vi "Command.vi"(8 "error in (no error)":errorcluster, 11 "Node Ptr":T1 format="%.0x") -> (0 "error out":errorcluster)   [LabVIEW 2020, in "Instrument Addon System Explorer.lvlib"]
uses:
  Instrument Addon System Explorer.lvlib
  <vilib>/NI VeriStand/Custom Device API/Custom Device API.lvlib
  Addon Shared/Instrument Addon Shared.lvlib
  Addon Shared/Types/FG Control.ctl
  <vilib>/NI VeriStand/Custom Device API/Custom Device Item Ref.ctl
panel:
  in  "Pad Value":u8=32 format="%.0x"
  in  "Length":u32=25 caption="Length (Bytes)"
  in  "Pad":bool caption="Pad?"
  in  "Linkages":i32(listbox)
  in  "MetaData":string(combo) caption="Available MetaData Channels"
  in  "Command":string caption="Command ( Use [] to define a variable )"
  in  "Header 2":cluster{"Section Name":string}={"Section Name"="Command Message Settings"}
  in  "SHDocVw.IWebBrowser":refnum<k7>(container)
  in  "Header":cluster{"Section Name":string}={"Section Name"="Command Settings"}
  in  "Description":string
  out "Name":string
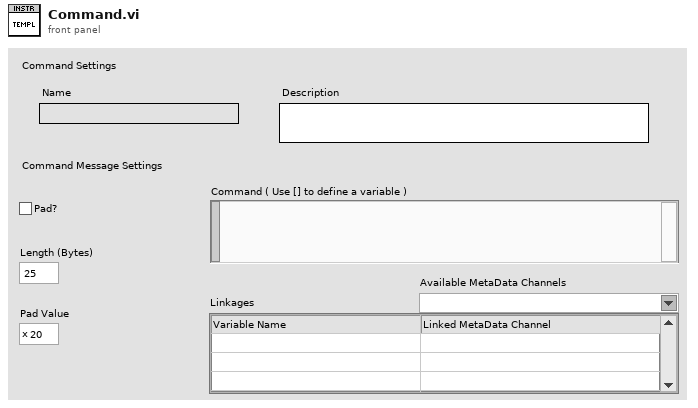
[diagram p1: front panel]
types:
  T1 = typedef "Custom Device API.lvlib/Custom Device Item Ref.ctl" = u64
  T2 = typedef "Instrument Addon Shared.lvlib/FG Control.ctl" = enum16{"Get", "Set"}
  T3 = typedef "Instrument Addon Shared.lvlib/Command Parameters.ctl" = cluster{"Command":string, "Linked Channels":T4[], "Pad":bool, "Length":u32, "Pad Value":u8}
  T4 = typedef "Instrument Addon Shared.lvlib/Linked Channel Cluster.ctl" = cluster{"Variable Name":string, "GUID":string}
  T5 = typedef "Custom Device API.lvlib/Custom Device Item Info.ctl" = cluster{"Name":string, "Is Channel":bool, "GUID":string, "Is Waveform":bool}
  T6 = typedef "Custom Device API.lvlib/Custom Device Commands.ctl" = enum16{"Default", "Item renamed", "Shutdown", "Dynamic button pressed"}
  T7 = typedef "LVComboBoxStrsAndValuesArrayTypeDef.ctl" = cluster{"String":string, "Value":string}[]
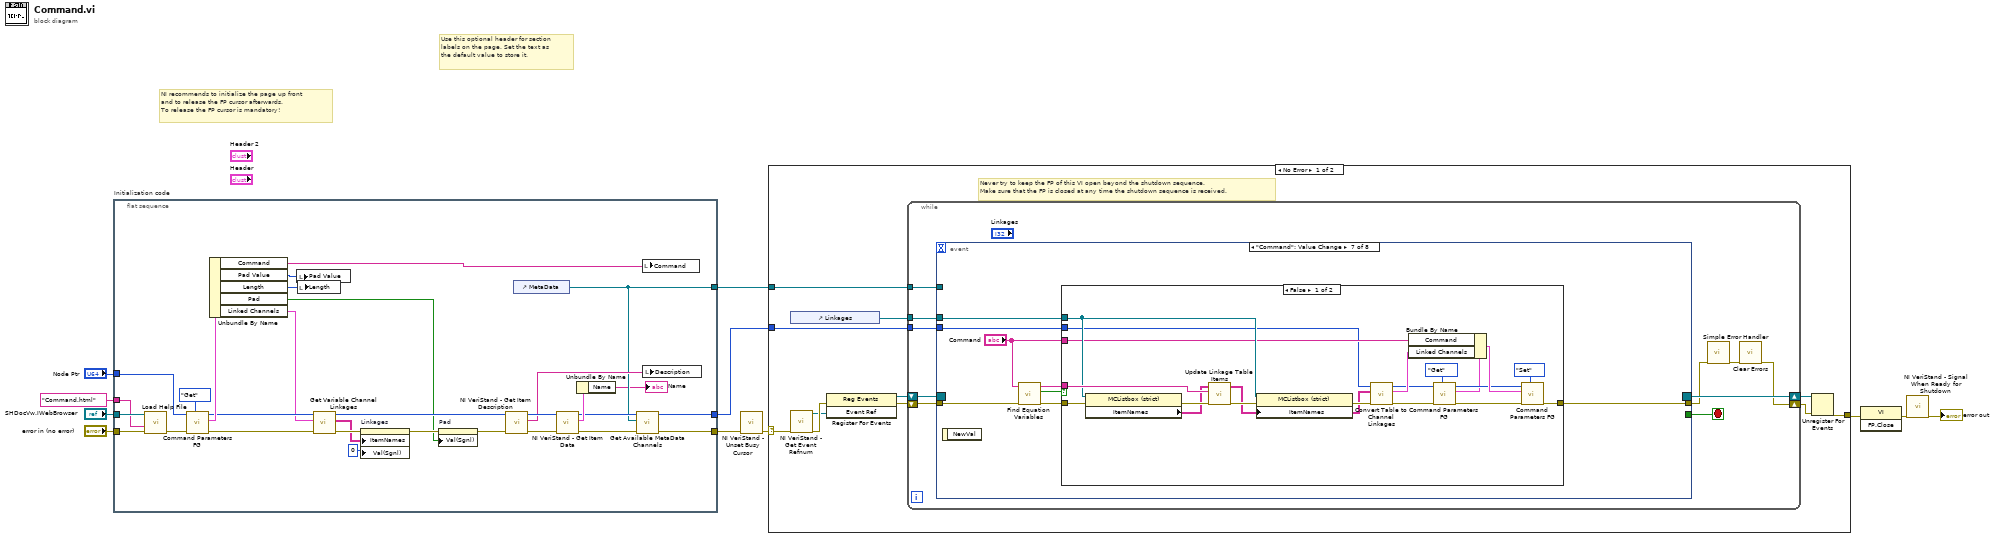
[diagram p0: block diagram]
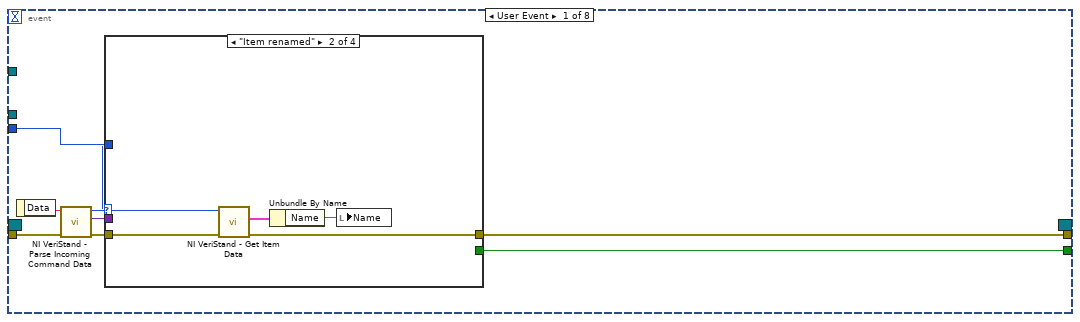
[diagram p2: hidden frame]
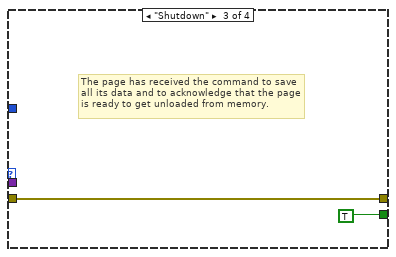
[diagram p4: hidden frame]
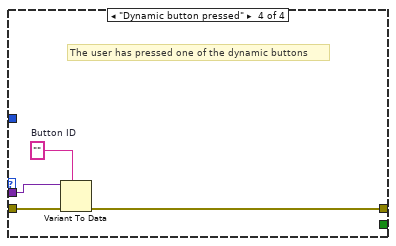
[diagram p5: hidden frame]
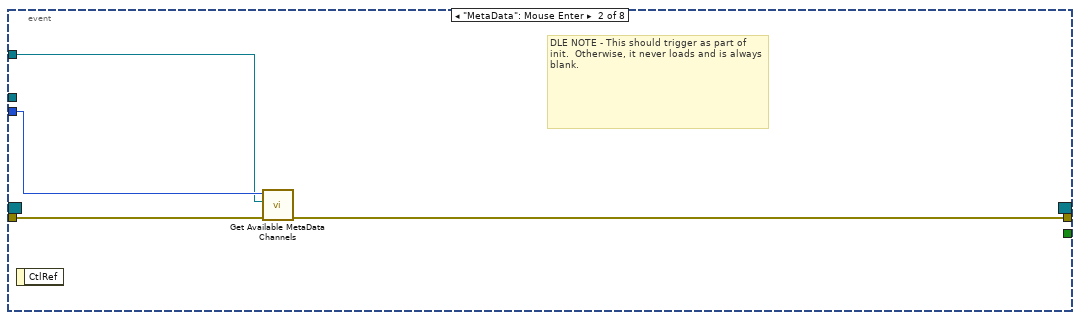
[diagram p6: hidden frame]
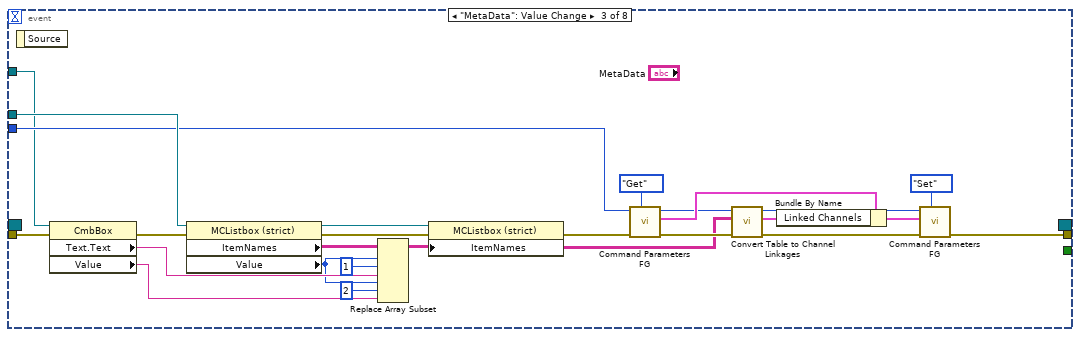
[diagram p7: hidden frame]
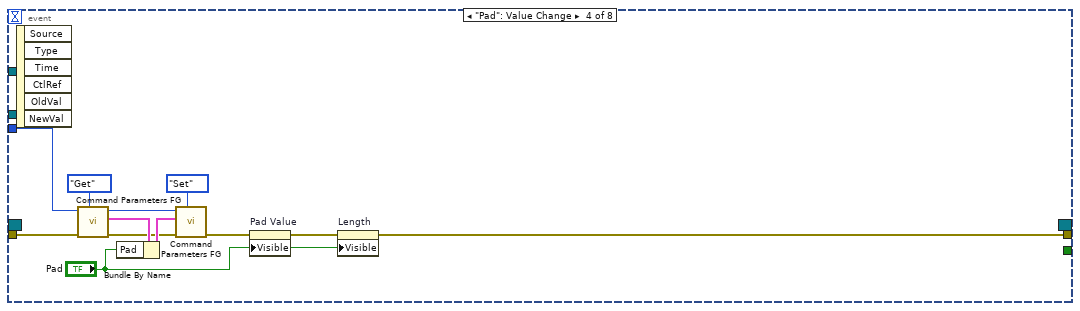
[diagram p8: hidden frame]
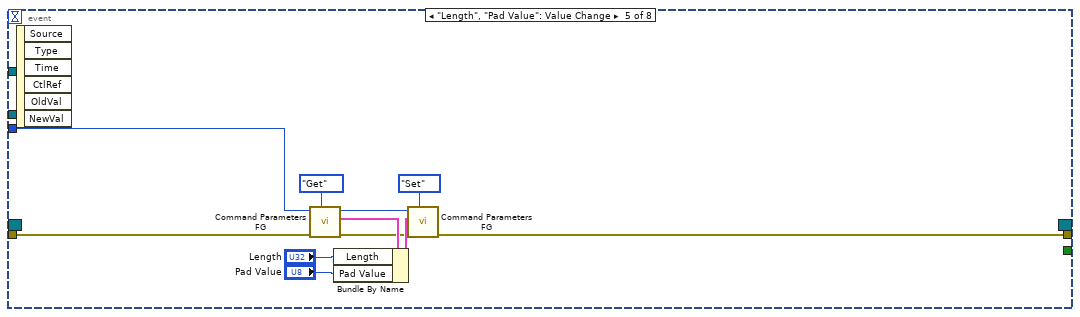
[diagram p9: hidden frame]
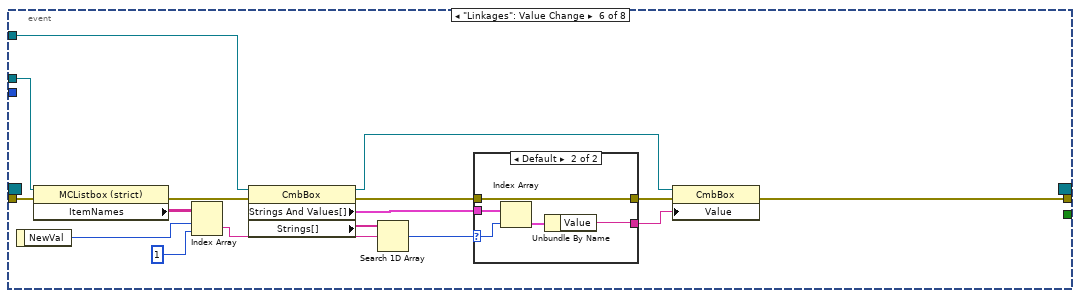
[diagram p10: hidden frame]
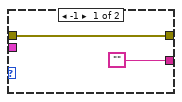
[diagram p11: hidden frame]
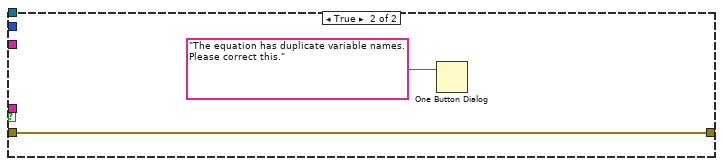
[diagram p12: hidden frame]
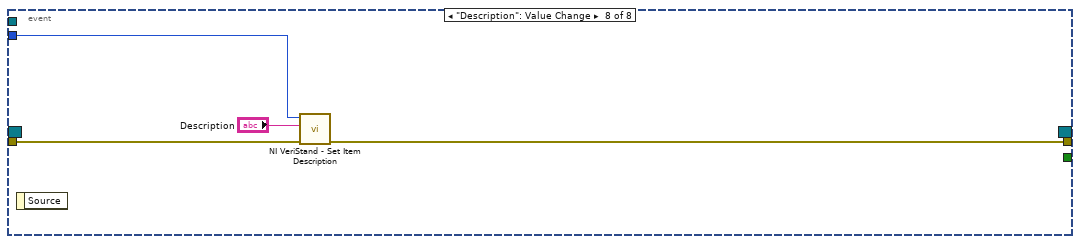
[diagram p13: hidden frame]
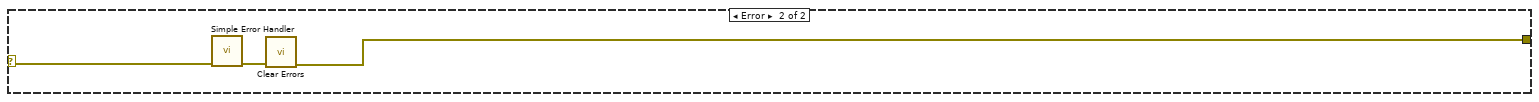
[diagram p14: hidden frame]
diagram:
  # "Use this optional header for section labels on the page. Set the text as the default value to store it."
  # "NI recommends to initialize the page up front\nand to release the FP cursor afterwards.\nTo release the FP cursor is mandatory!"
  n1 = flat-sequence "Initialization code" {
    tunnel: "error in (no error)" -> [w37]
    tunnel: "Node Ptr" -> [w33]
    tunnel: [w27] -> w7
    tunnel: [w25] -> w4
    tunnel: "SHDocVw.IWebBrowser" -> [w36]
    tunnel: "Command.html" ("HTML File") -> [w35]
    tunnel: [w24] -> w1
    frame #0 {
      n2 = call "Load Help File.vi"("error in (no error)"=w37, "HTML File to Load"=w35, "SHDocVw.IWebBrowser2"=w36) -> ("error out"=w32:errorcluster)  [unwired: 8 in]
      n3 = call "Command Parameters FG.vi"("Action"=FG_Control."Get", "error in (no error)"=w32, "Item Ref in"=w33) -> ("error out"=w22:errorcluster, "Command Parameters"=w31:T3, "Item Ref out"=w21:T1)  [unwired: 6 in]
      n4 = Unbundle By Name(w31) -> ("Command"=w30:string, "Pad Value"=w13:u8, "Length"=w12:u32, "Pad"=w14:bool, "Linked Channels"=w20:T4[])
      n5 = local write "Pad Value"(w13) -> ()
      n6 = local write "Length"(w12) -> ()
      n7 = call "Get Variable Channel Linkages.vi"("error in (no error)"=w22, "Linked Channels"=w20, "Item Ref in"=w21) -> ("error out"=w19:errorcluster, "Array"=w18:string[][], "Item Ref out"=w17:T1)  [unwired: 6 in]
      n8 = property on="Linkages" class="MCListbox (strict)"(error in=w19, "ItemNames"=w18, "Val(Sgnl)"=0 ("Value (Signaling)")) -> (error out=w16:errorcluster)  [unwired: 1 in, 1 out]
      n9 = property on="Pad" class="Bool (strict)"(error in=w16, "Val(Sgnl)"=w14) -> (error out=w15:errorcluster)  [unwired: 1 in, 1 out]
      n10 = call <vilib>:"NI VeriStand - Get Item Description.vi"("error in (no error)"=w15, "Item Ref in"=w17) -> ("error out"=w39:errorcluster, "Description"=w40:string, "Item Ref out"=w41:T1)  [unwired: 7 out]
      n11 = control-ref of="MetaData"() -> (w24:refnum<vi>)
      n12 = call <vilib>:"NI VeriStand - Get Item Data.vi"("error in (no error)"=w39, "Item Ref in"=w41) -> ("error out"=w28:errorcluster, "Item Info"=w38:T5, "Item Ref out"=w26:T1)  [unwired: 7 out]
      n13 = Unbundle By Name(w38) -> ("Name"=→"Name":string)
      n14 = call "Get Available MetaData Channels.vi"("error in (no error)"=w28, "MetaData"=w24, "Item Ref in"=w26) -> ("error out"=w27:errorcluster, "Item Ref out"=w25:T1)  [unwired: 7 in]
      n15 = local write "Command"(w30) -> ()
      n16 = local write "Description"(w40) -> ()
    }
  }
  n17 = call <vilib>:"NI VeriStand - Unset Busy Cursor.vi"("error in (no error)"=w7) -> ("error out"=w6:errorcluster)  [unwired: 10 out]
  n18 = case shown="No Error" w6 {
    selector: w6 -> [w44 w194]
    tunnel: [w49 w192] -> w11
    tunnel: w4 -> [w45 _]
    tunnel: w1 -> [w42 _]
    frame No Error {
      # "Never try to keep the FP of this VI open beyond the shutdown sequence.\nMake sure that the FP is closed at any time the shutdown sequence is received."
      n19 = call <vilib>:"NI VeriStand - Get Event Refnum.vi"("error in (no error)"=w44) -> ("error out"=w52:errorcluster, "Event Ref"=w48:refnum<user-event>)  [unwired: 9 out]
      n20 = control-ref of="Linkages"() -> (w43:refnum<vi>)
      n21 = register-events(error in=w52, w48) -> (reference out=w46:refnum<event-registration>, error out=w47:errorcluster)  [unwired: 1 in]
      n22 = while {
        tunnel: w45 -> [w54]
        shift-right: [w57] -> w50
        shift-left: w47 -> [w61]
        shift-right: [w62] -> w51
        shift-left: w46 -> [w60]
        tunnel: w43 -> [w56]
        tunnel: w42 -> [w55]
        stop <- w59 stop-if-true
        n23 = event shown="[6] \"Command\": Value Change" {
          selector: w60 -> [_ _ _ _ _ _ _ _]
          dyn-events: [_ _ _ _ _ _ _ _] -> w62
          timeout: _ -> [_ _ _ _ _ _ _ _]
          tunnel: w61 -> [w70 w86 w95 w118 w129 w150 w164 w190]
          tunnel: [w66 _ _ _ _ _ _ _] -> w59
          tunnel: [w65 w85 w103 w113 w126 w140 w161 w189] -> w53
          tunnel: w56 -> [_ _ w111 _ _ w149 w162 _]
          tunnel: w55 -> [_ w83 w96 _ _ w145 _ _]
          tunnel: w54 -> [w64 w84 w99 w120 w131 _ w159 w191]
          event User Event {
            n24 = event-data() -> ("Data"=w69:string)  [unwired: 1 out]
            n25 = call <vilib>:"NI VeriStand - Parse Incoming Command Data.vi"("error in (no error)"=w70, "Incoming data"=w69) -> ("error out"=w68:errorcluster, "Outgoing data"=w63:variant, "Action"=w67:T6)  [unwired: 7 out]
            n26 = case shown="\"Item renamed\"" w67 {
              tunnel: w68 -> [w71 w76 w77 w82]
              tunnel: [_ _ TRUE _] -> w66
              tunnel: [w71 w73 w77 w79] -> w65
              tunnel: w64 -> [_ w75 _ _]
              tunnel: w63 -> [_ _ _ w81]
              frame "Default", Default {
              }
              frame "Item renamed" {
                n27 = call <vilib>:"NI VeriStand - Get Item Data.vi"("error in (no error)"=w76, "Item Ref in"=w75) -> ("error out"=w73:errorcluster, "Item Info"=w74:T5)  [unwired: 8 out]
                n28 = Unbundle By Name(w74) -> ("Name"=w72:string)
                n29 = local write "Name"(w72) -> ()
              }
              frame "Shutdown" {
                # "The page has received the command to save all its data and to acknowledge that the page is ready to get unloaded from memory."
              }
              frame "Dynamic button pressed" {
                w80 = ""  # Button ID
                # "The user has pressed one of the dynamic buttons"
                n30 = Variant To Data(error in=w82, type=w80, Variant=w81) -> (error out=w79:errorcluster)  [unwired: 1 out]
              }
            }
          }
          event "MetaData": Mouse Enter {
            # "DLE NOTE - This should trigger as part of init.  Otherwise, it never loads and is always blank."
            n31 = event-data() -> ()  [unwired: 2 out]
            n32 = call "Get Available MetaData Channels.vi"("error in (no error)"=w86, "MetaData"=w83, "Item Ref in"=w84) -> ("error out"=w85:errorcluster)  [unwired: 7 in, 1 out]
          }
          event "MetaData": Value Change {
            n33 = event-data() -> ()  [unwired: 2 out]
            n34 = property class="CmbBox"(reference=w96, error in=w95) -> (error out=w94:errorcluster, "Text.Text"=w93:string, "Value"=w91:string)  [unwired: 1 out]
            n35 = property class="MCListbox (strict)"(reference=w111, error in=w94) -> (reference out=w108:refnum<vi>, error out=w107:errorcluster, "ItemNames"=w110:string[][], "Value"=w92:i32)
            n36 = Replace Array Subset(array=w110, new element #1=w93, index (row) #1=w92, index (col) #1=1 ("disabled index (col)"), new element #2=w91, index (row) #2=w92, index (col) #2=2 ("disabled index (col)")) -> (w90:string[][])
            n37 = property class="MCListbox (strict)"(reference=w108, error in=w107, "ItemNames"=w90) -> (error out=w101:errorcluster)  [unwired: 1 out]
            n38 = call "Command Parameters FG.vi"("Action"=FG_Control."Get", "error in (no error)"=w101, "Item Ref in"=w99) -> ("error out"=w100:errorcluster, "Command Parameters"=w98:T3, "Item Ref out"=w88:T1)  [unwired: 6 in]
            n39 = call "Convert Table to Channel Linkages.vi"("error in (no error)"=w100, "Item Names"=w90, "Item Ref in"=w88) -> ("error out"=w105:errorcluster, "Linkages"=w89:T4[], "Item Ref out"=w87:T1)  [unwired: 6 in]
            n40 = Bundle By Name(cluster=w98, "Linked Channels"=w89) -> (w104:T3)
            n41 = call "Command Parameters FG.vi"("Action"=FG_Control."Set", "error in (no error)"=w105, "Command Parameters"=w104, "Item Ref in"=w87) -> ("error out"=w103:errorcluster)  [unwired: 5 in, 2 out]
          }
          event "Pad": Value Change {
            n42 = event-data() -> ()  [unwired: 7 out]
            n43 = call "Command Parameters FG.vi"("Action"=FG_Control."Get", "error in (no error)"=w118, "Item Ref in"=w120) -> ("error out"=w117:errorcluster, "Command Parameters"=w119:T3, "Item Ref out"=w116:T1)  [unwired: 6 in]
            n44 = Bundle By Name(cluster=w119, "Pad"="Pad") -> (w122:T3)
            n45 = call "Command Parameters FG.vi"("Action"=FG_Control."Set", "error in (no error)"=w117, "Command Parameters"=w122, "Item Ref in"=w116) -> ("error out"=w114:errorcluster)  [unwired: 5 in, 2 out]
            n46 = property on="Pad Value" class="DigNum (strict)"(error in=w114, "Visible"="Pad") -> (error out=w115:errorcluster)  [unwired: 1 in, 1 out]
            n47 = property on="Length" class="DigNum (strict)"(error in=w115, "Visible"="Pad") -> (error out=w113:errorcluster)  [unwired: 1 in, 1 out]
          }
          event "Length", "Pad Value": Value Change {
            n48 = event-data() -> ()  [unwired: 7 out]
            n49 = call "Command Parameters FG.vi"("Action"=FG_Control."Get", "error in (no error)"=w129, "Item Ref in"=w131) -> ("error out"=w128:errorcluster, "Command Parameters"=w130:T3, "Item Ref out"=w127:T1)  [unwired: 6 in]
            n50 = Bundle By Name(cluster=w130, "Length"="Length", "Pad Value"="Pad Value") -> (w133:T3)
            n51 = call "Command Parameters FG.vi"("Action"=FG_Control."Set", "error in (no error)"=w128, "Command Parameters"=w133, "Item Ref in"=w127) -> ("error out"=w126:errorcluster)  [unwired: 5 in, 2 out]
          }
          event "Linkages": Value Change {
            n52 = event-data() -> ("NewVal"=w147:i32)  [unwired: 1 out]
            n53 = property class="MCListbox (strict)"(reference=w149, error in=w150) -> (error out=w144:errorcluster, "ItemNames"=w148:string[][])  [unwired: 1 out]
            n54 = Index Array(array=w148, index (row)=w147, index (col)=1 ("disabled index (col)")) -> (element=w143:string)
            n55 = property class="CmbBox"(reference=w145, error in=w144) -> (reference out=w138:refnum<vi>, error out=w136:errorcluster, "Strings And Values[]"=w142:T7, "Strings[]"=w135:string[])
            n56 = Search 1D Array(1D array=w135, element=w143) -> (index of element=w139:i32)  [unwired: 1 in]
            n57 = case shown="Default" w139 {
              selector: w139 -> [_ w155]
              tunnel: w142 -> [_ w157]
              tunnel: ["" w153] -> w141
              tunnel: [w152 w154] -> w137
              tunnel: w136 -> [w152 w154]
              frame -1 {
              }
              frame Default {
                n58 = Index Array(array=w157, index=w155) -> (element=w156:cluster{"String":string, "Value":string})
                n59 = Unbundle By Name(w156) -> ("Value"=w153:string)
              }
            }
            n60 = property class="CmbBox"(reference=w138, error in=w137, "Value"=w141) -> (error out=w140:errorcluster)  [unwired: 1 out]
          }
          event "Command": Value Change {
            n61 = event-data() -> ()  [unwired: 2 out]
            n62 = call "Find Equation Variables.vi"("error in (no error)"=w164, "Command"="Command") -> ("error out"=w163:errorcluster, "Duplicate?"=w158:bool, "Variables"=w165:string[])  [unwired: 7 in]
            n63 = case shown="False" w158 {
              tunnel: w165 -> [w185 _]
              tunnel: w163 -> [w184 w187]
              tunnel: w162 -> [w180 _]
              tunnel: [w179 w187] -> w161
              tunnel: "Command" -> [w178 _]
              tunnel: w159 -> [w172 _]
              frame False {
                n64 = property class="MCListbox (strict)"(reference=w180, error in=w184) -> (error out=w183:errorcluster, "ItemNames"=w182:string[][])  [unwired: 1 out]
                n65 = call "Update Linkage Table Items.vi"("error in (no error)"=w183, "Variables"=w185, "Item Names"=w182) -> ("error out"=w181:errorcluster, "Item Names"=w174:string[][])  [unwired: 7 in]
                n66 = property class="MCListbox (strict)"(reference=w180, error in=w181, "ItemNames"=w174) -> (error out=w176:errorcluster)  [unwired: 1 out]
                n67 = call "Convert Table to Channel Linkages.vi"("error in (no error)"=w176, "Item Names"=w174, "Item Ref in"=w172) -> ("error out"=w170:errorcluster, "Linkages"=w173:T4[], "Item Ref out"=w168:T1)  [unwired: 6 in]
                n68 = call "Command Parameters FG.vi"("Action"=FG_Control."Get", "error in (no error)"=w170, "Item Ref in"=w168) -> ("error out"=w169:errorcluster, "Command Parameters"=w166:T3, "Item Ref out"=w167:T1)  [unwired: 6 in]
                n69 = Bundle By Name(cluster=w166, "Command"=w178, "Linked Channels"=w173) -> (w175:T3)
                n70 = call "Command Parameters FG.vi"("Action"=FG_Control."Set", "error in (no error)"=w169, "Command Parameters"=w175, "Item Ref in"=w167) -> ("error out"=w179:errorcluster)  [unwired: 5 in, 2 out]
              }
              frame True {
                n71 = One Button Dialog(message="The equation has duplicate variable names.  Please correct this.") -> ()  [unwired: 1 in, 1 out]
              }
            }
          }
          event "Description": Value Change {
            n72 = event-data() -> ()  [unwired: 2 out]
            n73 = call <vilib>:"NI VeriStand - Set Item Description.vi"("error in (no error)"=w190, "Description"="Description", "Item Ref in"=w191) -> ("error out"=w189:errorcluster)  [unwired: 8 out]
          }
        }
        n74 = call <vilib>:"Simple Error Handler.vi"("error in (no error)"=w53) -> ("error out"=w58:errorcluster)  [unwired: 1 in, 7 out]
        n75 = call <vilib>:"Clear Errors.vi"("error in (no error)"=w58) -> ("error out"=w57:errorcluster)  [unwired: 1 in, 5 out]
      }
      n76 = Unregister For Events(event registration refnum=w51, error in=w50) -> (error out=w49:errorcluster)
    }
    frame Error {
      n77 = call <vilib>:"Simple Error Handler.vi"("error in (no error)"=w194) -> ("error out"=w193:errorcluster)  [unwired: 1 in, 7 out]
      n78 = call <vilib>:"Clear Errors.vi"("error in (no error)"=w193) -> ("error out"=w192:errorcluster)  [unwired: 1 in, 5 out]
    }
  }
  n79 = invoke class="VI" method="FP.Close"(error in=w11) -> (error out=w10:errorcluster)  [unwired: 2 in, 2 out]
  n80 = call <vilib>:"NI VeriStand - Signal When Ready for Shutdown.vi"("error in (no error)"=w10) -> ("error out"=→"error out":errorcluster)  [unwired: 10 out]
